vi "to_json.vi"(8 "error in":errorcluster, 11 "labels in":refnum<class "labels.lvclass">) -> (0 "error out":errorcluster, 2 "json":string, 3 "labels out":refnum<class "labels.lvclass">, 4 "Not Default":bool)   [LabVIEW 2020, in "nominal types.lvlib" / "labels.lvclass"]
uses:
  labels.lvclass
  labels.lvclass/labels.ctl
  cab77863-f927-4ae1-98ba-0267e36df10e.vi
  b8486177-9344-4009-9026-0c4df4e1a446.vi
  <vilib>/JDP Science/JSONtext/Variant to JSON Text.vi
  <vilib>/JDP Science/JSONtext/LVClass Serializer/JSONtext LVClass Serializer.lvclass
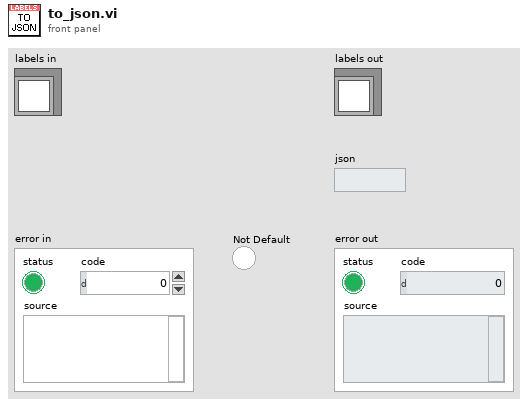
[diagram p1: front panel]
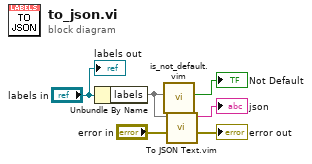
[diagram p0: block diagram]
diagram:
  n1 = Unbundle By Name("labels in") -> ("labels"=w2:set{string})
  n2 = call "is_not_default.vim"("data"=w2) -> ("Not Default"=→"Not Default":bool)  [unwired: 10 in]
  n3 = call "To JSON Text.vim"("error in (no error)"="error in", "Anything"=w2) -> ("error out"=→"error out":errorcluster, "<JSON>"=→"json":string)  [unwired: 8 in]
  "labels out" <- "labels in"
